vi "Get Font .NET.vi"(11 "Font in":refnum<class "Font.lvclass">) -> (2 "Font .NET":refnum<k24>, 3 "Font out":refnum<class "Font.lvclass">)   [LabVIEW 2020, in "SourceGrid.lvlib" / "Font.lvclass"]
uses:
  Font.lvclass
  System.Drawing
  Font.lvclass/Font.ctl
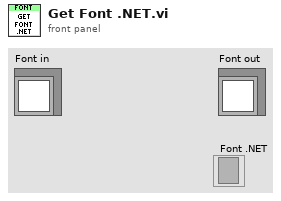
[diagram p1: front panel]
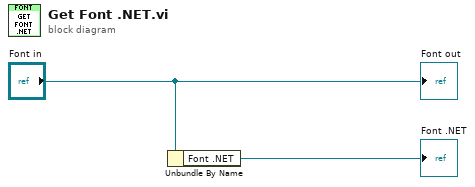
[diagram p0: block diagram]
diagram:
  n1 = Unbundle By Name("Font in") -> ("Font .NET"=→"Font .NET":refnum<k24>)
  "Font out" <- "Font in"
